vi "test Get-Set-Get Parameter Definitions.vi"(8 "error in":errorcluster, 11 "TestCase in":refnum<class "Scripting.lvclass">) -> (0 "error out":errorcluster, 3 "TestCase out":refnum<class "Scripting.lvclass">)   [LabVIEW 2020, in "Scripting.lvclass"]
uses:
  Scripting.lvclass
  Scripting.lvclass/Scripting.ctl
  C:/Program Files/National Instruments/LabVIEW 2026/vi.lib/addons/_JKI Toolkits/VI Tester/TestCase.llb/TestCase.lvclass
  C:/git/fmussi_niveristand-aim-arinc429-custom-device/Source/Custom Device Support/Tests/Unit/Scripting/Scripting.lvclass
  <vilib>/addons/_JKI Toolkits/VI Tester/TestCase.llb/TestCase.lvclass
  Scripting/AIM/AIM ARINC 429 Scripting.lvlib
  <vilib>/NI/NI VeriStand Encoding and Decoding/Encoding.ctl
  <vilib>/NI/NI VeriStand Encoding and Decoding/Encoding and Decoding.lvlib
  Shared/Parameter Definition.ctl
  Shared/Direction.ctl
  Shared/SDI.ctl
  Shared/Transfer Type.ctl
  Shared/Transfer Speed.ctl
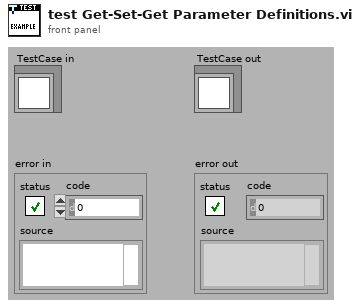
[diagram p1: front panel]
types:
  T1 = typedef "Transfer Speed.ctl" = enum16{"LO (12.5 kb/s)", "HI (100 kb/s)"}
  T2 = typedef "Transfer Type.ctl" = enum16{"Scheduled", "Acyclic", "Block", "Strobe"}
  T3 = typedef "Direction.ctl" = enum16{"Rx", "Tx"}
  T4 = typedef "SDI.ctl" = i32
  T5 = typedef "Parameter Definition.ctl" = cluster{"start index":i32, "size":i32, "encoding":T6, "signed":bool, "scale multiplier":dbl, "scale offset":dbl, "default value":dbl}
  T6 = typedef "Encoding and Decoding.lvlib/Encoding.ctl" = enum16{"BNR", "BCD", "Discrete"}
  T7 = typedef "Custom Device API.lvlib/Custom Device Item Ref.ctl" = u64
  T8 = typedef "Custom Device API.lvlib/Custom Device Channel.ctl" = cluster{"Type":T9, "Units":string, "Default Value":dbl, "Faultable":bool, "Scalable":bool}
  T9 = typedef "Custom Device API.lvlib/Custom Device Channel Type.ctl" = enum16{"Input", "Output"}
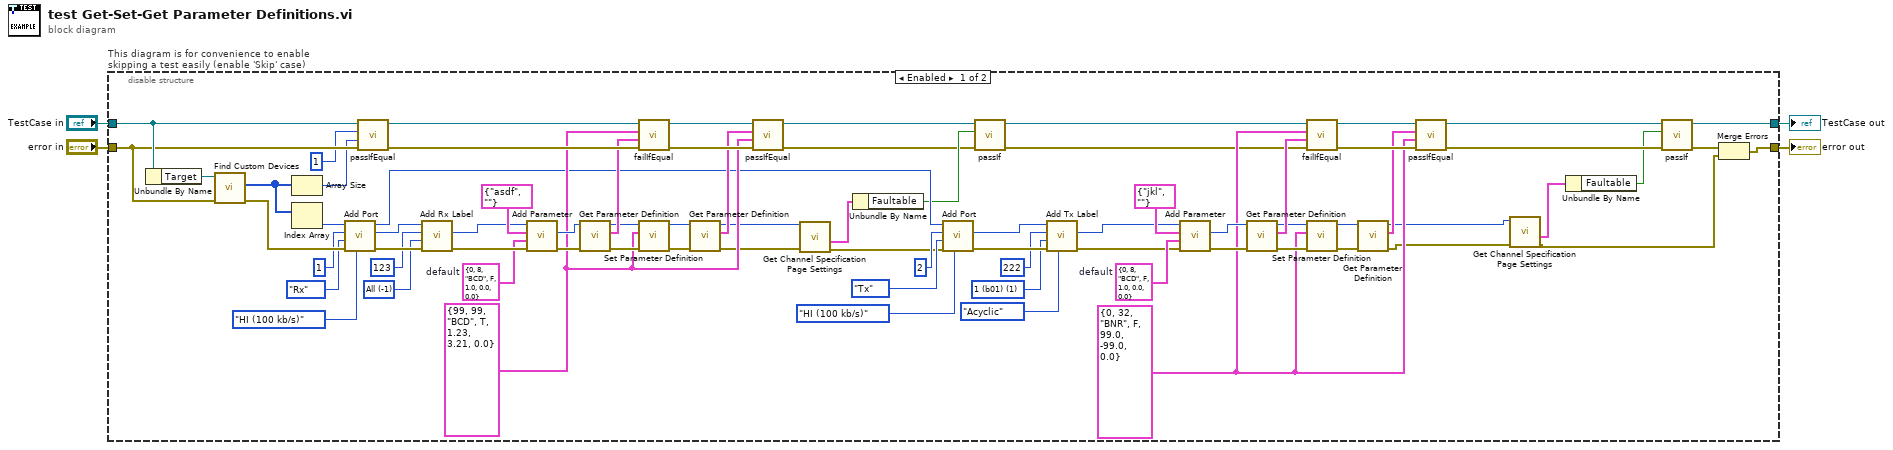
[diagram p0: block diagram]
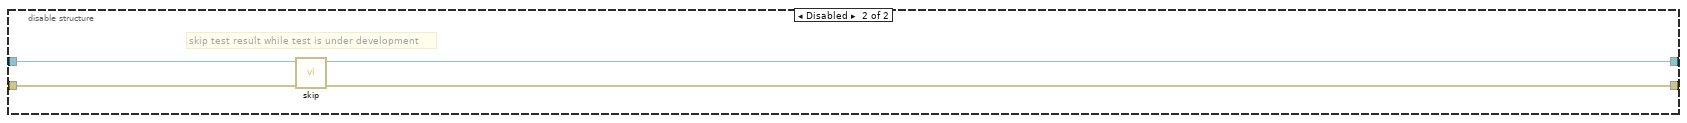
[diagram p2: hidden frame]
diagram:
  n1 = disable-structure "This diagram is for convenience to enable skipping a test easily (enable 'Skip' case)" shown="Enabled" {
    disable-tunnel: "TestCase in" -> [w78 w83]
    disable-tunnel: [w7 w81] -> w1
    disable-tunnel: [w72 w82] -> w3
    disable-tunnel: "error in" -> [w77 w80]
    frame Enabled {
      w29 = T4 1 items=["All"=-1, "0 (b00)"=0, "1 (b01)"=1, "2 (b10)"=2, "3 (b11)"=3] ("SDI value")
      w39 = T5 {"start index"=0, "size"=8, "encoding"=enum."BCD", "signed"=FALSE, "scale multiplier"=1.0, "scale offset"=0.0, "default value"=0.0}  # default
      w42 = T5 {"start index"=0, "size"=8, "encoding"=enum."BCD", "signed"=FALSE, "scale multiplier"=1.0, "scale offset"=0.0, "default value"=0.0}  # default
      w47 = T4 -1 items=["All"=-1, "0 (b00)"=0, "1 (b01)"=1, "2 (b10)"=2, "3 (b11)"=3] ("SDI value")
      w40 = T5 {"start index"=99, "size"=99, "encoding"=enum."BCD", "signed"=TRUE, "scale multiplier"=1.23, "scale offset"=3.21, "default value"=0.0} ("parameter definition")
      w33 = T5 {"start index"=0, "size"=32, "encoding"=enum."BNR", "signed"=FALSE, "scale multiplier"=99.0, "scale offset"=-99.0, "default value"=0.0} ("parameter definition")
      n2 = Unbundle By Name(w78) -> ("Target"=w79:refnum<k24>)
      n3 = call "Find Custom Devices.vi"("error in"=w77, "target"=w79) -> ("error out"=w55:errorcluster, "AIM ARINC 429 custom devices"=w57:T7[])  [unwired: 7 in, 1 out]
      n4 = Array Size(array=w57) -> (size(s)=w75:i32)
      n5 = Index Array(array=w57) -> (element=w56:T7)  [unwired: 1 in]
      n6 = call "Add Port.vi"("speed"=Transfer_Speed."HI (100 kb/s)", "error in"=w55, "direction"=Direction."Rx", "port number"=u16 1, "custom device ref"=w56) -> ("error out"=w49:errorcluster, "port"=w50:T7, "custom device ref out"=w28:T7)  [unwired: 4 in]
      n7 = call-dynamic "passIfEqual.vi"("error in (no error)"=w77, "y"=w75, "x"=1 ("size(s)"), "TestCase in"=w78) -> ("error out"=w73:errorcluster, "TestCase out"=w74:refnum<class "Scripting.lvclass">)  [unwired: 6 in]
      n8 = call "Add Rx Label.vi"("error in"=w49, "SDI value"=w47, "label value"=u32 123, "port ref"=w50) -> ("error out"=w45:errorcluster, "label"=w26:T7)  [unwired: 5 in, 1 out]
      n9 = call "Add Parameter.vi"("error in"=w45, "parameter encoding"=w42, "parameter definition"=cluster{"name":string, "unit":string} {"name"="asdf", "unit"=""}, "label ref"=w26) -> ("error out"=w43:errorcluster, "parameter"=w44:T7)  [unwired: 5 in, 1 out]
      n10 = call "Get Parameter Definition.vi"("error in"=w43, "parameter ref"=w44) -> ("error out"=w69:errorcluster, "parameter definition"=w70:T5, "parameter ref out"=w68:T7)  [unwired: 7 in]
      n11 = call-dynamic "failIfEqual.vi"("error in (no error)"=w73, "y"=w70, "x"=w40, "TestCase in"=w74) -> ("error out"=w65:errorcluster, "TestCase out"=w64:refnum<class "Scripting.lvclass">)  [unwired: 6 in]
      n12 = call "Set Parameter Definition.vi"("error in"=w69, "parameter definition"=w40, "parameter ref"=w68) -> ("error out"=w67:errorcluster, "parameter ref out"=w66:T7)  [unwired: 7 in]
      n13 = call "Get Parameter Definition.vi"("error in"=w67, "parameter ref"=w66) -> ("error out"=w22:errorcluster, "parameter definition"=w41:T5, "parameter ref out"=w20:T7)  [unwired: 7 in]
      n14 = call-dynamic "passIfEqual.vi"("error in (no error)"=w65, "y"=w40, "x"=w41, "TestCase in"=w64) -> ("error out"=w16:errorcluster, "TestCase out"=w17:refnum<class "Scripting.lvclass">)  [unwired: 6 in]
      n15 = call "Get Channel Specification Page Settings.vi"("error in"=w22, "parameter ref"=w20) -> ("error out"=w21:errorcluster, "Channel"=w19:T8)  [unwired: 6 in, 2 out]
      n16 = Unbundle By Name(w19) -> ("Faultable"=w18:bool)
      n17 = call "Add Port.vi"("speed"=Transfer_Speed."HI (100 kb/s)", "error in"=w21, "direction"=Direction."Tx", "port number"=u16 2, "custom device ref"=w28) -> ("error out"=w37:errorcluster, "port"=w36:T7)  [unwired: 4 in, 1 out]
      n18 = call-dynamic "passIf.vi"("error in (no error)"=w16, "pass"=w18, "TestCase in"=w17) -> ("error out"=w15:errorcluster, "TestCase out"=w14:refnum<class "Scripting.lvclass">)  [unwired: 7 in]
      n19 = call "Add Tx Label.vi"("transfer type"=Transfer_Type."Acyclic", "error in"=w37, "SDI value"=w29, "label value"=u32 222, "port ref"=w36) -> ("error out"=w31:errorcluster, "label"=w25:T7)  [unwired: 4 in, 1 out]
      n20 = call "Add Parameter.vi"("error in"=w31, "parameter encoding"=w39, "parameter definition"=cluster{"name":string, "unit":string} {"name"="jkl", "unit"=""}, "label ref"=w25) -> ("error out"=w35:errorcluster, "parameter"=w34:T7)  [unwired: 5 in, 1 out]
      n21 = call "Get Parameter Definition.vi"("error in"=w35, "parameter ref"=w34) -> ("error out"=w61:errorcluster, "parameter definition"=w71:T5, "parameter ref out"=w60:T7)  [unwired: 7 in]
      n22 = call-dynamic "failIfEqual.vi"("error in (no error)"=w15, "y"=w71, "x"=w33, "TestCase in"=w14) -> ("error out"=w59:errorcluster, "TestCase out"=w58:refnum<class "Scripting.lvclass">)  [unwired: 6 in]
      n23 = call "Set Parameter Definition.vi"("error in"=w61, "parameter definition"=w33, "parameter ref"=w60) -> ("error out"=w62:errorcluster, "parameter ref out"=w63:T7)  [unwired: 7 in]
      n24 = call "Get Parameter Definition.vi"("error in"=w62, "parameter ref"=w63) -> ("error out"=w13:errorcluster, "parameter definition"=w32:T5, "parameter ref out"=w11:T7)  [unwired: 7 in]
      n25 = call-dynamic "passIfEqual.vi"("error in (no error)"=w59, "y"=w33, "x"=w32, "TestCase in"=w58) -> ("error out"=w9:errorcluster, "TestCase out"=w8:refnum<class "Scripting.lvclass">)  [unwired: 6 in]
      n26 = call "Get Channel Specification Page Settings.vi"("error in"=w13, "parameter ref"=w11) -> ("error out"=w12:errorcluster, "Channel"=w10:T8)  [unwired: 6 in, 2 out]
      n27 = Unbundle By Name(w10) -> ("Faultable"=w5:bool)
      n28 = call-dynamic "passIf.vi"("error in (no error)"=w9, "pass"=w5, "TestCase in"=w8) -> ("error out"=w6:errorcluster, "TestCase out"=w7:refnum<class "Scripting.lvclass">)  [unwired: 7 in]
      n29 = Merge Errors(w6, w12) -> (w72:errorcluster)
    }
    frame Disabled {
      # "skip test result while test is under development"
      n30 = call <vilib>:"skip.vi"("error in (no error)"=w80, "TestCase in"=w83) -> ("error out"=w82:errorcluster, "TestCase out"=w81:refnum<class "Scripting.lvclass">)  [unwired: 8 in]
    }
  }
  "error out" <- w3
  "TestCase out" <- w1
